vi "Save Image.vi"(8 "error in":errorcluster, 9 "Measurements":dbl[][](array[numeric]), 10 "Sample name":string, 11 "base path":path) -> (0 "error out":errorcluster)   [LabVIEW 2021]
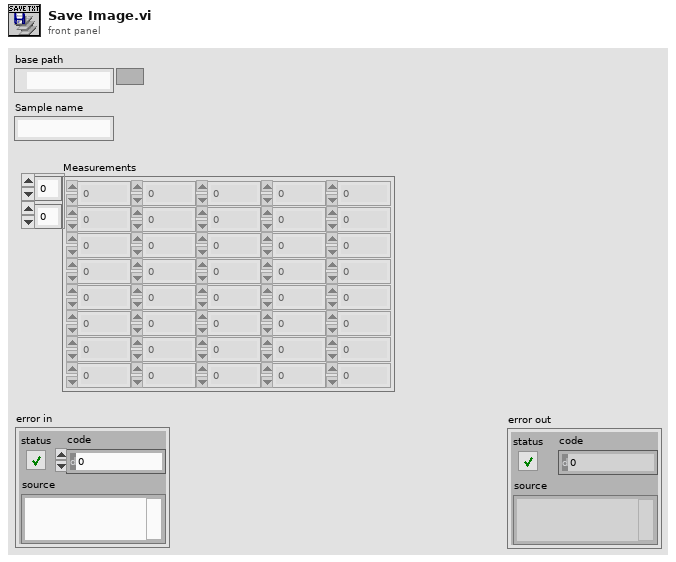
[diagram p1: front panel]
types:
  T1 = enum16{"open", "replace", "create", "open or create", "replace or create", "replace or create with confirmation"}
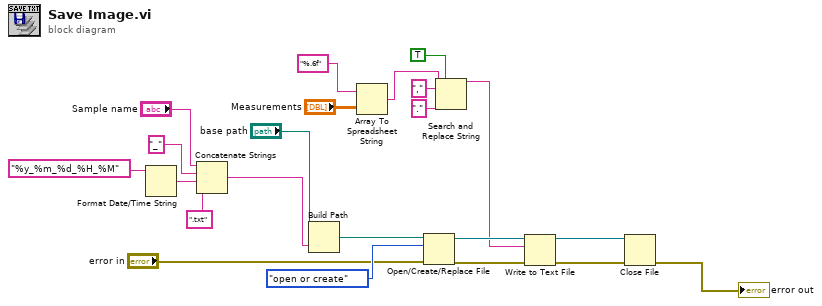
[diagram p0: block diagram]
diagram:
  n1 = Format Date/Time String(time format string (%c)="%y_%m_%d_%H_%M") -> (date/time string=w20:string)  [unwired: 2 in]
  n2 = Concatenate Strings("Sample name", "_" ("string"), w20, ".txt" ("string")) -> (w4:string)
  n3 = Build Path(base path="base path", name or relative path=w4) -> (appended path=w16:path)
  n4 = Array To Spreadsheet String(array="Measurements", 3:"%.6f" ("format string")) -> (spreadsheet string=w3:string)  [unwired: 1 in]
  n5 = Open/Create/Replace File(file path (use dialog)=w16, error in="error in", operation (0:open)=T1."open or create") -> (refnum out=w11:refnum<file>, error out=w15:errorcluster)  [unwired: 3 in, 1 out]
  n6 = Search and Replace String(replace all?=TRUE ("replace all? (F)"), input string=w3, search string=",", replace string="." ("replace string (\"\")")) -> (result string=w2:string)  [unwired: 4 in, 3 out]
  n7 = Write to Text File(file (use dialog)=w11, text=w2, error in=w15) -> (refnum out=w10:refnum<file>, error out=w14:errorcluster)  [unwired: 1 in, 1 out]
  n8 = Close File(refnum=w10, error in=w14) -> (error out=→"error out":errorcluster)  [unwired: 1 out]
